vi "VIH HelpGen - Save Image.vi"(5 "HTML Folder":path, 6 "BG Color (default)":u32(colorbox)=16777215, 7 "Image Folder":path, 8 "error in":errorcluster, 9 "Always overwrite (F)":bool, 10 "Image Filename":string, 11 "image data":T1) -> (0 "error out":errorcluster, 1 "HTML tag":string, 2 "path for HTML":string)   [LabVIEW 2014]
doc: "::: VI Helpeks :::\nCopyright (c) 2000-2026 Konstantin Shifershteyn. All rights reserved."
uses:
  <vilib>/picture/picture.llb/imagedata.ctl
panel:
  # "VI Helpeks\nCopyright (c) 2012-2026 Konstantin Shifershteyn"
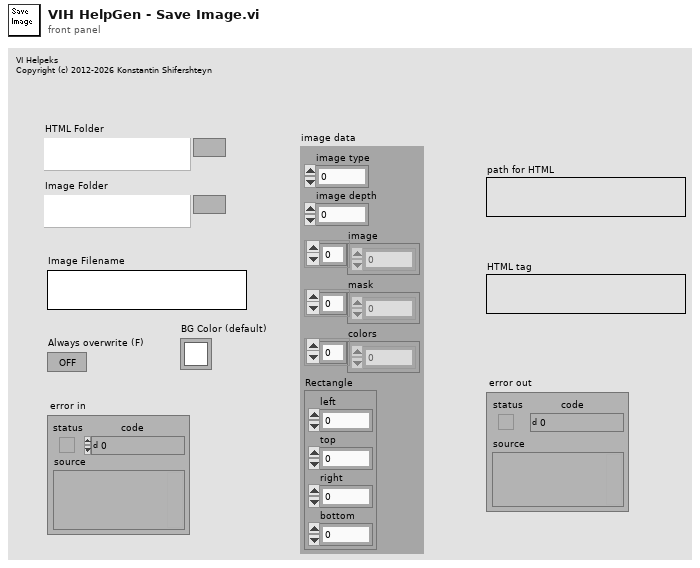
[diagram p1: front panel]
types:
  T1 = typedef "imagedata.ctl" = cluster{"image type":i32, "image depth":i32, "image":u8[], "mask":u8[], "colors":u32[], "Rectangle":cluster{"left":i16, "top":i16, "right":i16, "bottom":i16}}
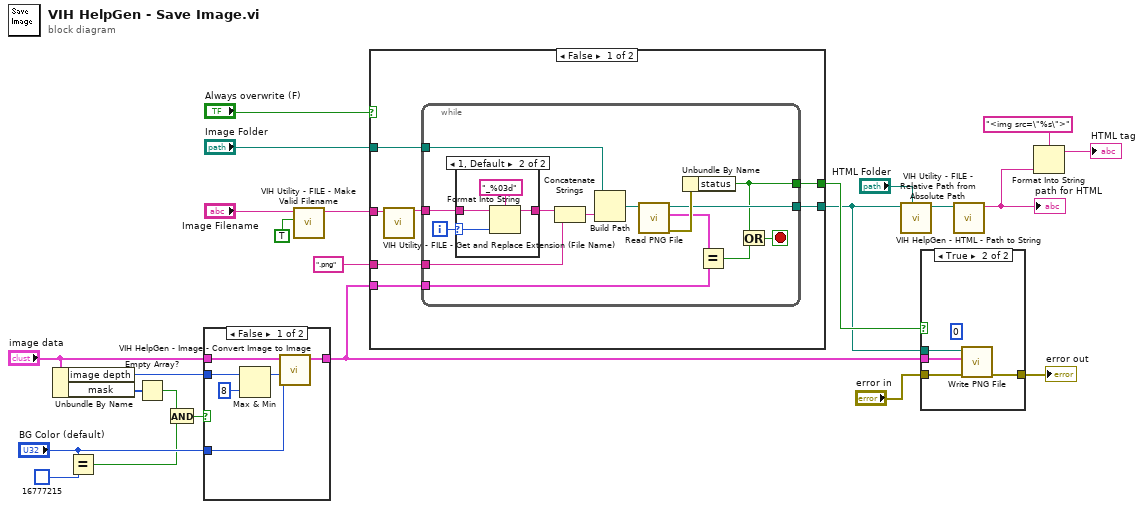
[diagram p0: block diagram]
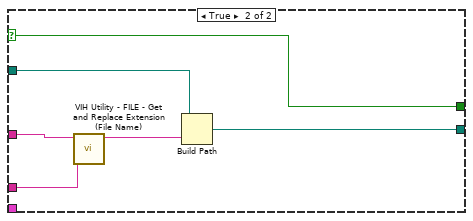
[diagram p4: hidden frame]
diagram:
  n1 = Unbundle By Name("image data") -> ("image depth"=w7:i32, "mask"=w8:u8[])
  n2 = Equal?(x="BG Color (default)", y=u32 16777215 ("BG Color (white)")) -> (x = y?=w4:bool)
  n3 = Empty Array?(array=w8) -> (empty?=w3:bool)
  n4 = And(x=w3, y=w4) -> (x .and. y?=w2:bool)
  n5 = case shown="False" w2 {
    tunnel: "image data" -> [w30 w31]
    tunnel: [w29 w31] -> w9
    tunnel: w7 -> [w27 _]
    tunnel: "BG Color (default)" -> [w25 _]
    frame False {
      n6 = Max & Min(x=w27, y=8) -> (max(x,y)=w28:i32)  [unwired: 1 out]
      n7 = call "VIH HelpGen - Image - Convert Image to Image.vi"("BG Color (white)"=w25, "color depth (as source)"=w28, "image data"=w30) -> ("image data out"=w29:T1)  [unwired: 8 in]
    }
    frame True {
    }
  }
  n8 = call "VIH Utility - FILE - Make Valid Filename.vi"("comply to CHM (F)"=TRUE, "File Name in"="Image Filename") -> ("File Name out"=w18:string)  [unwired: 9 in]
  n9 = case shown="False" "Always overwrite (F)" {
    selector: "Always overwrite (F)" -> [_ w58]
    tunnel: "Image Folder" -> [w38 w60]
    tunnel: w9 -> [w37 _]
    tunnel: [w36 w59] -> w11
    tunnel: [w35 w58] -> w19
    tunnel: w18 -> [w34 w62]
    tunnel: ".png" ("new extension (none)") -> [w32 w63]
    frame False {
      n10 = call "VIH Utility - FILE - Get and Replace Extension (File Name).vi"("File name"=w34) -> ("File name out"=w33:string)  [unwired: 9 in, 1 out]
      n11 = while {
        tunnel: w38 -> [w52]
        tunnel: w33 -> [w50]
        tunnel: [w45] -> w36
        tunnel: w37 -> [w44]
        tunnel: [w42] -> w35
        tunnel: w32 -> [w41]
        i -> [w49]
        stop <- w43 stop-if-true
        n12 = case shown="1, Default" w49 {
          selector: w49 -> [_ w55]
          tunnel: w50 -> [w53 w57]
          tunnel: [w53 w54] -> w48
          frame 0 {
          }
          frame 1, Default {
            n13 = Format Into String(format string="_%03d", initial string=w57, w55) -> (resulting string=w54:string)  [unwired: 1 in, 1 out]
          }
        }
        n14 = Concatenate Strings(w48, w41) -> (w51:string)
        n15 = Build Path(base path=w52, name or relative path=w51) -> (appended path=w47:path)
        n16 = call <vilib>:"Read PNG File.vi"("path to PNG file"=w47) -> ("error out"=w46:errorcluster, "image data"=w40:T1, "path"=w45:path)  [unwired: 8 in]
        n17 = Unbundle By Name(w46) -> ("status"=w42:bool)
        n18 = Equal?(x=w40, y=w44) -> (x = y?=w39:bool)
        n19 = Or(x=w42, y=w39) -> (x .or. y?=w43:bool)
      }
    }
    frame True {
      n20 = call "VIH Utility - FILE - Get and Replace Extension (File Name).vi"("new extension (none)"=w63, "File name"=w62) -> ("File name out"=w61:string)  [unwired: 8 in, 1 out]
      n21 = Build Path(base path=w60, name or relative path=w61) -> (appended path=w59:path)
    }
  }
  n22 = call "VIH Utility - FILE - Relative Path from Absolute Path.vi"("base path (empty: dir of Top VI)"="HTML Folder", "Path"=w11) -> ("Rel Path out"=w15:path)  [unwired: 7 in, 2 out]
  n23 = case shown="True" w19 {
    tunnel: [w64 w68] -> w23
    tunnel: w9 -> [_ w65]
    tunnel: w11 -> [_ w67]
    tunnel: "error in" -> [w64 w66]
    frame False {
    }
    frame True {
      (unwired) 0 ("compression (default)")
      n24 = call <vilib>:"Write PNG File.vi"("error in (no error)"=w66, "image data"=w65, "path to PNG file"=w67) -> ("error out"=w68:errorcluster)  [unwired: 7 in, 1 out]
    }
  }
  "error out" <- w23
  n25 = call "VIH HelpGen - HTML - Path to String.vi"("Path"=w15) -> ("String"=w13:string)  [unwired: 10 in]
  "path for HTML" <- w13
  n26 = Format Into String(format string="<img src=\"%s\">", w13) -> (resulting string=→"HTML tag":string)  [unwired: 2 in, 1 out]
